vi "Read Unpacked Files.vi"(8 "error in (no error)":errorcluster, 11 "PackageFile in":refnum<class "PackageFile.lvclass">) -> (0 "error out":errorcluster, 2 "Unpacked files":path[](array[path]), 3 "PackageFile out":refnum<class "PackageFile.lvclass">)   [LabVIEW 2020, in "vi_package_building_extensions.lvlib" / "PackageFile.lvclass"]
uses:
  PackageFile.lvclass
  PackageFile.lvclass/PackageFile.ctl
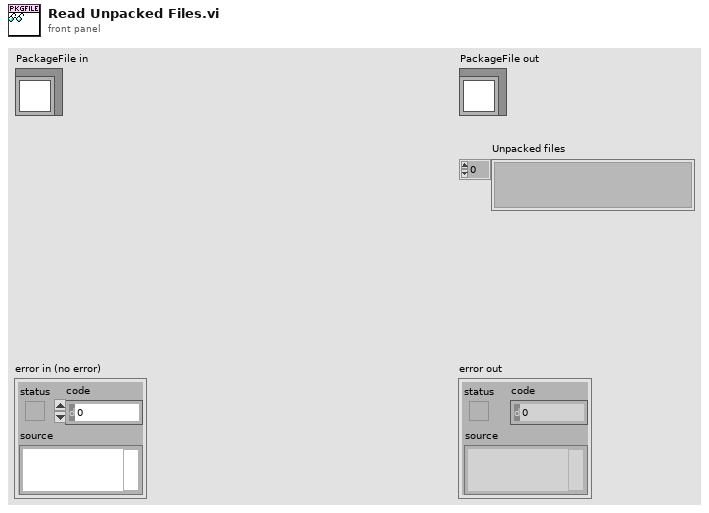
[diagram p1: front panel]
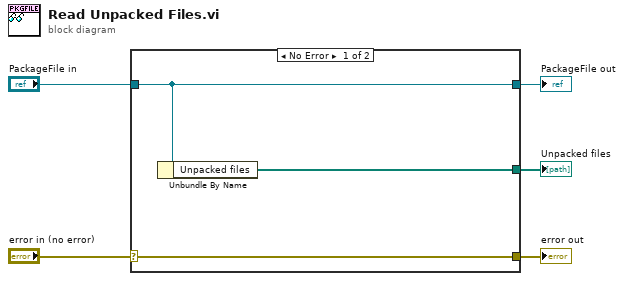
[diagram p0: block diagram]
diagram:
  n1 = case shown="No Error" "error in (no error)" {
    selector: "error in (no error)" -> [w8 w9]
    tunnel: [w8 w9] -> w4
    tunnel: [w7 w10] -> w2
    tunnel: "PackageFile in" -> [w7 w10]
    tunnel: [w6 _] -> w1
    frame No Error {
      n2 = Unbundle By Name(w7) -> ("Unpacked files"=w6:path[])
    }
    frame Error {
    }
  }
  "error out" <- w4
  "PackageFile out" <- w2
  "Unpacked files" <- w1
